vi "ZM-PC-getTypeName.vi"(8 "error in (no error)":errorcluster, 11 "ZM-PC-package in":refnum<class "ZM-PC-package.lvclass">) -> (0 "error out":errorcluster, 2 "type_name":string, 3 "ZM-PC-package out":refnum<class "ZM-PC-package.lvclass">)   [LabVIEW 2020, in "ZM-PC-packages.lvlib" / "ZM-PC-package.lvclass"]
doc: "Returns the name of the package type, i.e. the item name of the ZM-PC-PACKAGE_TYPE enum read through Read type (Undefined, TestPackage or ErrorPackage). The only VI the rest of the code uses to name a type."
uses:
  ZM-PC-package.lvclass
  ZM-PC-package.lvclass/ZM-PC-package.ctl
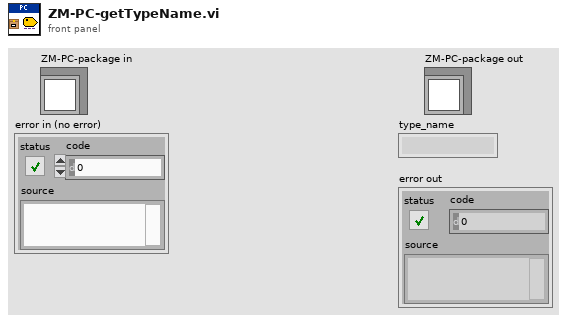
[diagram p1: front panel]
types:
  T1 = typedef "ZM-PC-packages.lvlib/ZM-PC-package.lvclass/ZM-PC-PACKAGE_TYPE.ctl" = enum16{"Undefined", "TestPackage", "ErrorPackage"}
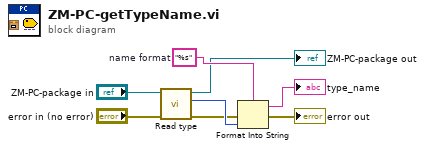
[diagram p0: block diagram]
diagram:
  w6 = "%s"  # name format
  n1 = call "Read type.vi"("error in (no error)"="error in (no error)", "ZM-PC-package in"="ZM-PC-package in") -> ("error out"=w4:errorcluster, "ZM-PC-PACKAGE_TYPE"=w5:T1, "ZM-PC-package out"=→"ZM-PC-package out":refnum<class "ZM-PC-package.lvclass">)  [unwired: 7 in]
  n2 = Format Into String(format string=w6, error in=w4, w5) -> (resulting string=→"type_name":string, error out=→"error out":errorcluster)  [unwired: 1 in]
